vi "Needle Valve labVIEW Code.vi"() -> ()   [LabVIEW 2025]
uses:
  PIDController/PIDController.lvclass
  spikeController/spikeController.lvclass
  ControllerModeEnum.ctl
  modesEnum.ctl
  PIDController/PIDController.lvclass/PIDController.ctl
  0285ecf2-4d18-4427-ace1-61b1951a0741.vi
  d3b0afdc-d7ac-4f1a-8ecc-0aeb21fe1e80.vi
  c8945bc9-af31-4a2e-9b52-27840c61c0f1.vi
  e7797c04-791b-4eea-89a1-5a3bec2431d3.vi
  bf5fd3a0-ddf8-478e-bb95-a39885d33854.vi
  0890acf7-df83-934e-a7ac-ae51bc85d557.vi
  d872897a-af24-4a4d-87bc-a1bb59a840a8.vi
  <vilib>/Instr/_visa.llb/VISA Configure Serial Port (Instr).vi
  PIDController/updateLastValues.vi
  <vilib>/Utility/file.llb/Write Delimited Spreadsheet (string).vi
  <vilib>/Utility/file.llb/Read Delimited Spreadsheet (DBL).vi
  <vilib>/gmath/NI_Gmath.lvlib
  <vilib>/ptbypt/NI_PtbyPt.lvlib
panel:
  out "Motor Response":string
  in  "Disconnect":bool
  in  "Connect":bool
  in  "Use Dummy Data":bool
  in  "Reset":bool
  out "Reading Pressure Sensor 2":dbl(graph)
  out "PID Output 2":dbl(graph)
  out "the setted point":dbl
  out "the set position":dbl
  out "auto k_d":dbl
  out "auto k_i":dbl
  out "auto k_p":dbl
  out "spike str":string
  out "Array-to-save Pressure":string[][](array[string])
  out "Array-to-save PID":string[][](array[string])
  out "Array-to-save Spike":string[][](array[string])
  out "Array-to-save":string[][](array[string])
  out "to save":path
  out "Time Elapsed":dbl
  out "cycles_run":i32
  out "Autotune":bool
  in  "dt":dbl
  in  "tuning_rule":i32
  in  "min_cycles":i32
  in  "hysteresis":dbl
  in  "relay_amplitude":dbl
  in  "Exit Autotune":bool
  in  "AutoTune PID Params":bool
  out "last error":dbl
  in  "Use D1":bool
  in  "Use D2":bool
  in  "Use Avg":bool
  in  "Save Graphs":bool
  in  "Set setPoint":dbl format="%.3f"
  in  "Set Spike Position":dbl format="%.3f"
  in  "setPoint":dbl(knob) scale=0.0..1000.0
  in  "A_max":dbl=6.5
  in  "A_min":dbl
  in  "k_i":dbl
  in  "k_d":dbl
  in  "k_p":dbl
  out "SafetyClose":bool
  out "PID":bool
  out "Manual":bool
  out "Idle":bool
  out "Ducer1":bool
  out "Ducer2":bool
  out "Avg Ducers":bool
  out "Read Pressure Ducer":dbl
  out "Raw Pressure Ducer 2":dbl
  in  "spikeController.lvclass":refnum<class "spikeController.lvclass">
  out "underAmin":bool
  out "overAmax":bool
  out "PID Output":dbl[](graph)
  out "PID Translated Output":dbl
  out "PID Raw Output":dbl
  in  "loop stop 2":bool
  in  "loop stop 1":bool
  in  "PIDController.lvclass":refnum<class "PIDController.lvclass">
  out "VISA resource name out":refnum<visa-resource-name>
  in  "?":u32(colorbox)=16777225
  out "Reading Pressure Sensor":dbl[](graph)
  in  "?":dbl
  out "Motor Signal":string
  in  "stop program":bool
  in  "return spike":bool
  out "Spike Position \n(via Potentiometer)":dbl[](graph)
  out "Arduino Error":errorcluster
  in  "VISA resource Port":refnum<visa-resource-name>
  out "distance to go":dbl caption="Distance to Go (in)\n(For Reference Only)" format="%.3f"
  out "spike position":dbl format="%.3f"
  in  "Set Spike Position (in)":dbl(slide) scale=0.1..6.6
  out "?":dbl(slide) scale=0.0..1000.0
  out "Stagnation Flow Temp (K)\n(For Refrence only)":dbl
  out "Raw Pressure Ducer":dbl
  in  "Sensor Offsets":dbl[](array[numeric])=[10.0, 10.0, 0.0, 22.0]
  in  "Sensor K-values":dbl[](array[numeric])=[10.0, 10.0, 0.0, 22.0]
  in  "Exit PID Mode":bool
  in  "manual exit button":bool
  in  "Motor Control Loop Rate (ms)":dbl
  out "Set Motor RPM":dbl(knob) scale=0.0..200.0
  in  "PID Mode":bool
  in  "Manual Positioning Mode":bool
  in  "Stop Sensors":bool
  in  "Sensor Loop Rate (ms)":dbl
  out "Time Since Start (s)\n(For Reference Only)":dbl format="%.2f"
  in  "Start Sensors":bool
  in  "Load Inputs":bool
  in  "Save Inputs":bool
  out "Potentiometer distance":dbl
  out "Port":i32
  out "ConnectionType":i32
  out "DeviceType":i32
  out "Labjack error":errorcluster
  # "34HS59-6004S Motor Torque Curve (For Reference)"
  # "Labjack/Arduino Resources"
  # "Inputs and LabJack Sensor Monitors"
  # "PID Inputs"
  # "Motor RPM >200 RPM"
  # "Potentiometer"
  # "Inefficent Torque for High Mass Flow/Thrust Tests"
  # "Ducer"
  # "Thermocouple"
  # "<-- Uses same setpoint"
  # "Motor RPM < 200 RPM"
  # "(Labjack Auto-Populates)"
  # "(dial indicator for range reference)"
  # "COM Port for Arduino"
  # "Stop sensors automatically saves sensor data"
  # "Needliest"
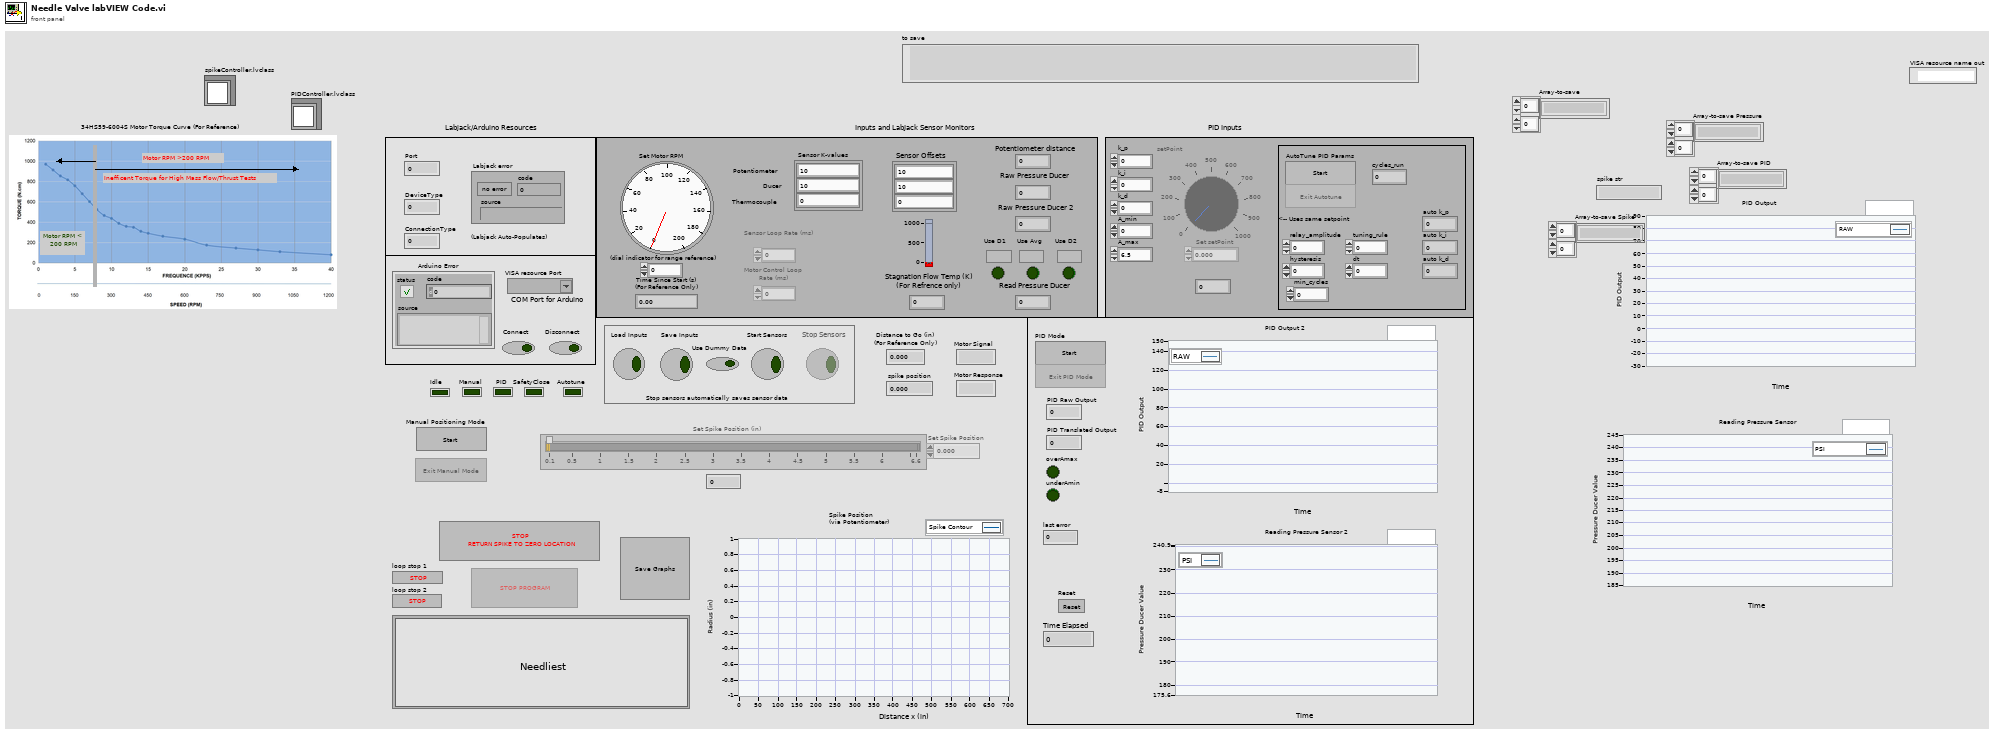
[diagram p1: front panel]
types:
  T1 = typedef "ControllerModeEnum.ctl" = enum16{"", "startControllers", "IdleControllers"}
  T2 = typedef "modesEnum.ctl" = enum16{"relay_autotune", "SafetyOpen", "SafetyClose", "SaveFile", "PIDControl", "ManualControl", "Idle"}
  T3 = enum8{"Enabled", "Disabled", "Disabled and Grayed Out"}
  T4 = enum16{"Potentiometer", "Ducer", "Thermocouple", "Ducer2"}
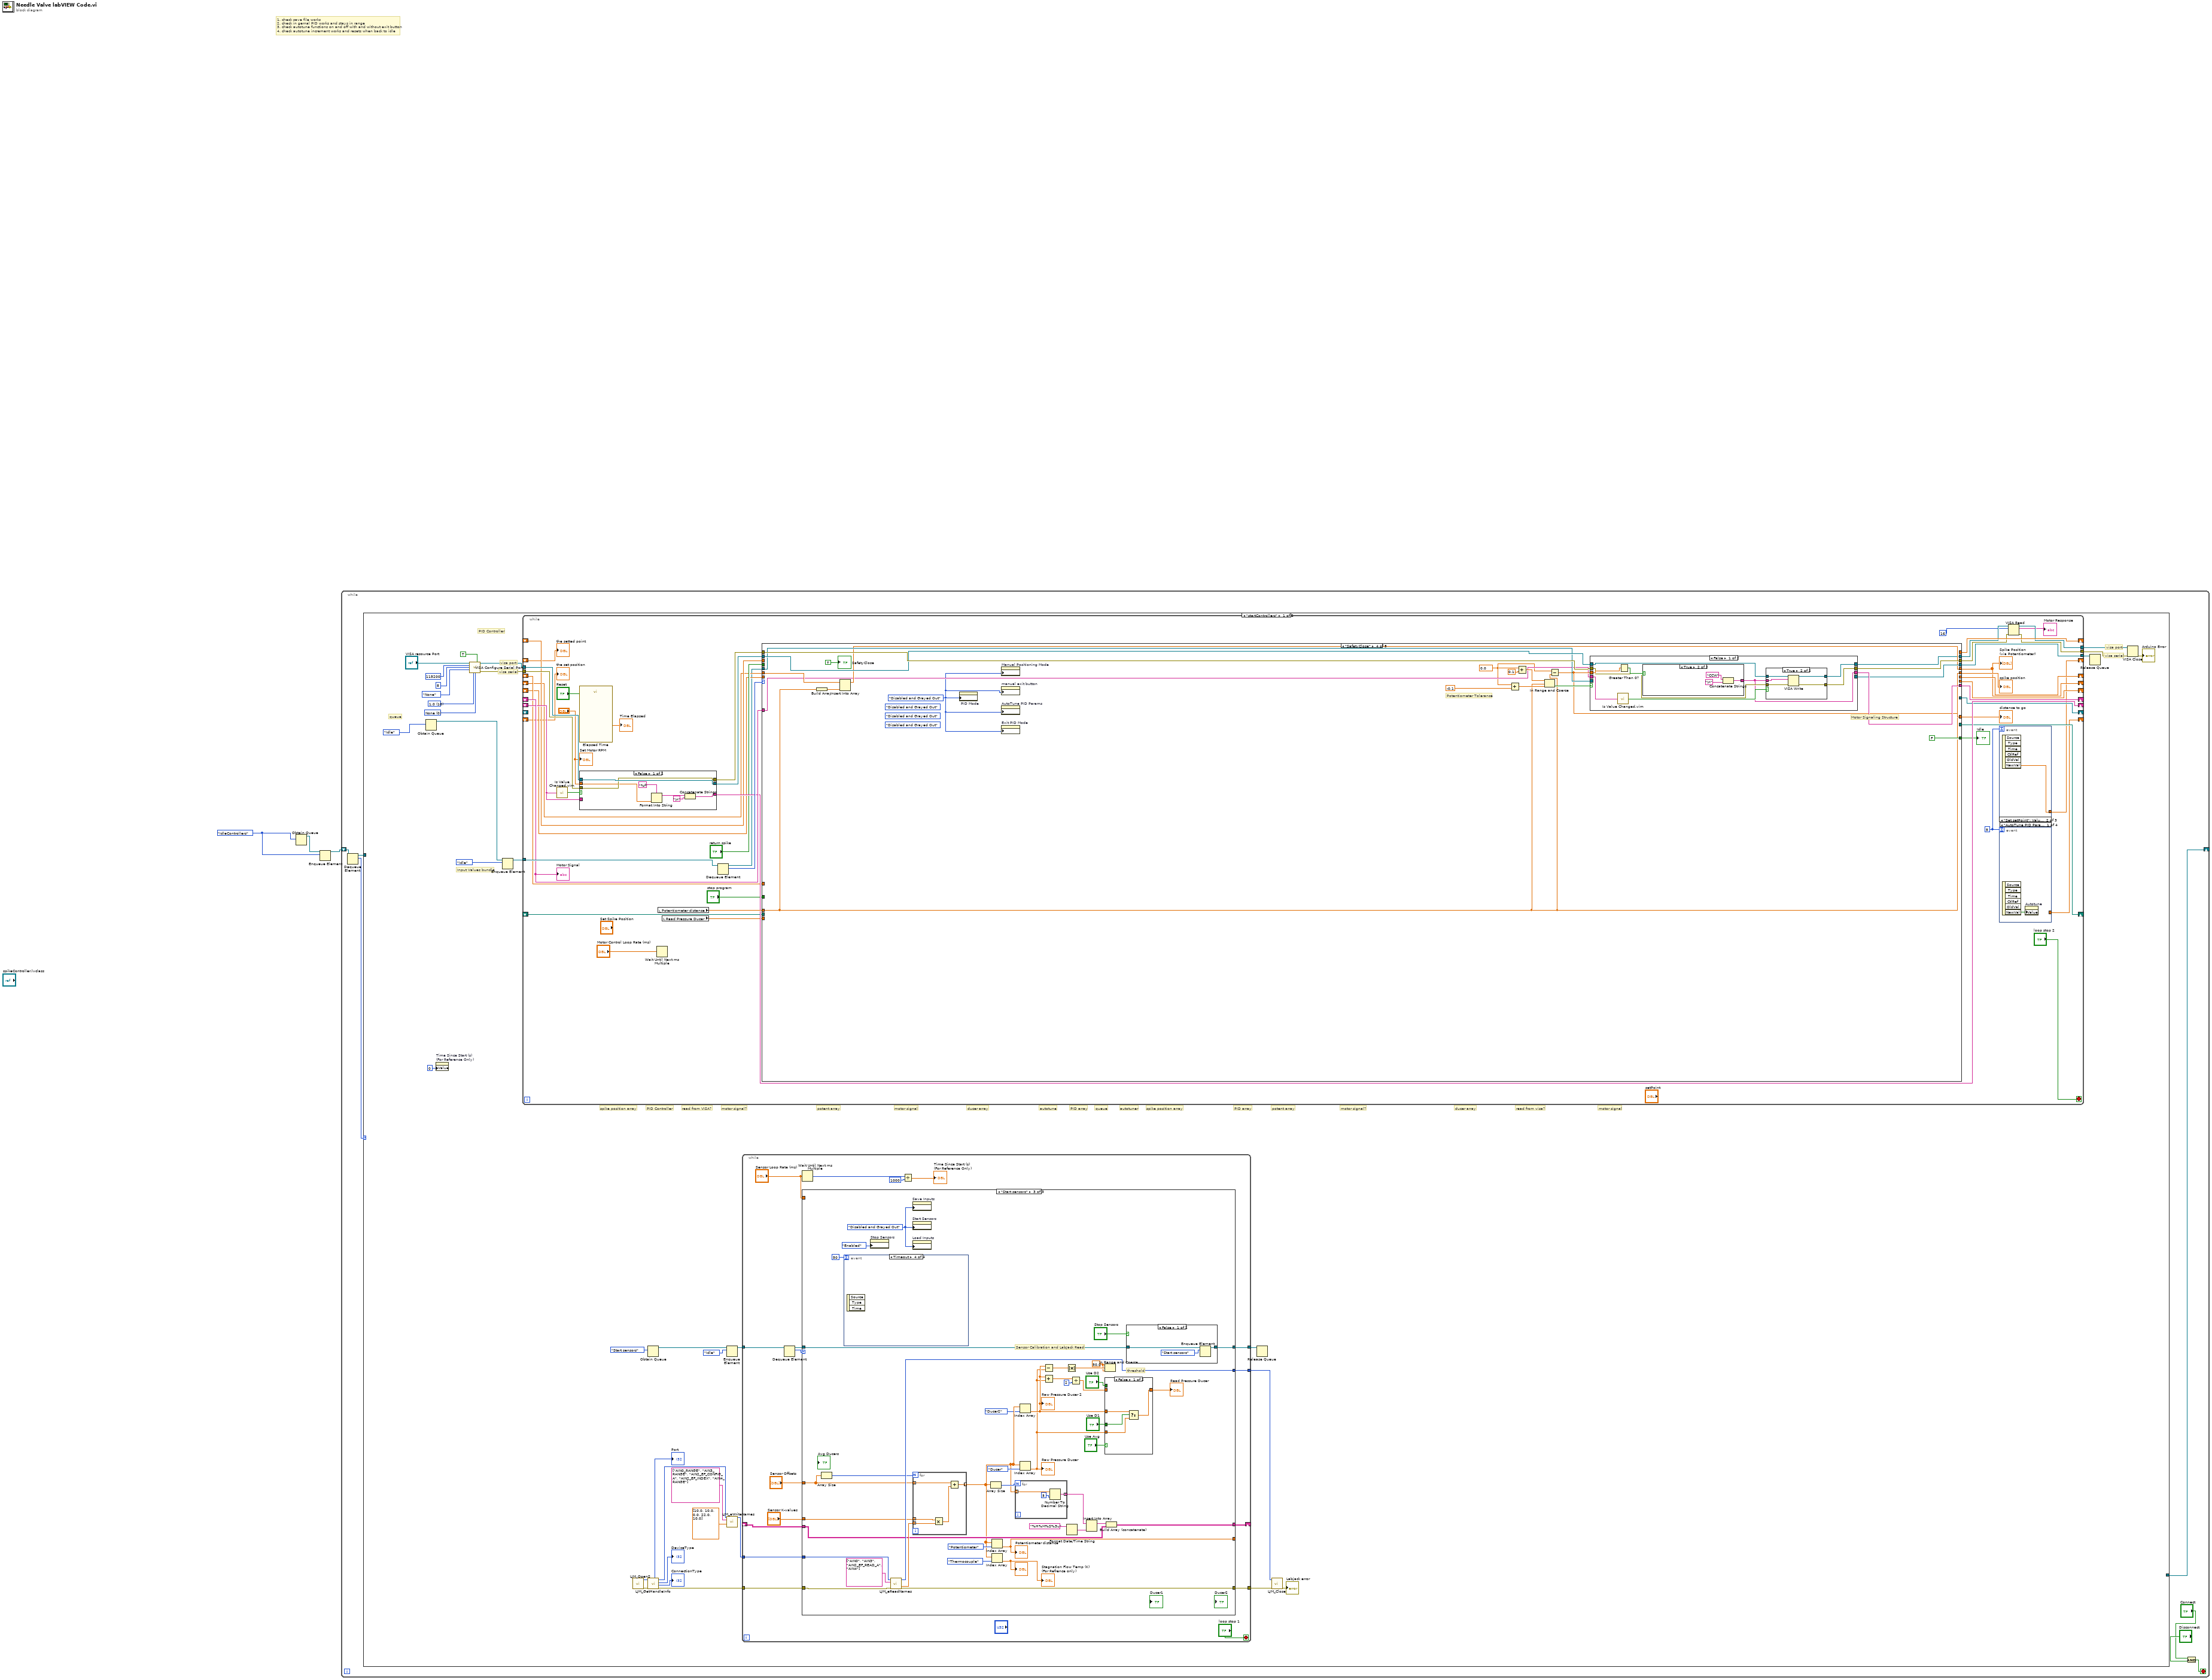
[diagram p0: block diagram]
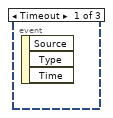
[diagram p2: hidden frame]
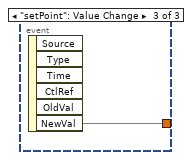
[diagram p3: hidden frame]
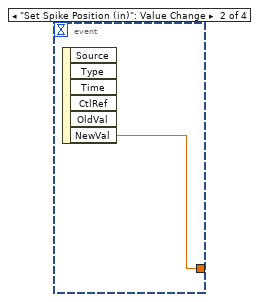
[diagram p4: hidden frame]
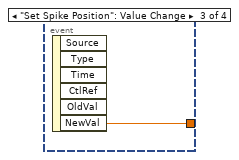
[diagram p5: hidden frame]
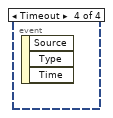
[diagram p6: hidden frame]
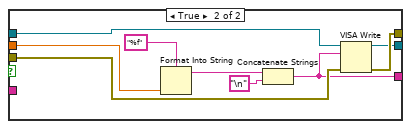
[diagram p7: hidden frame]
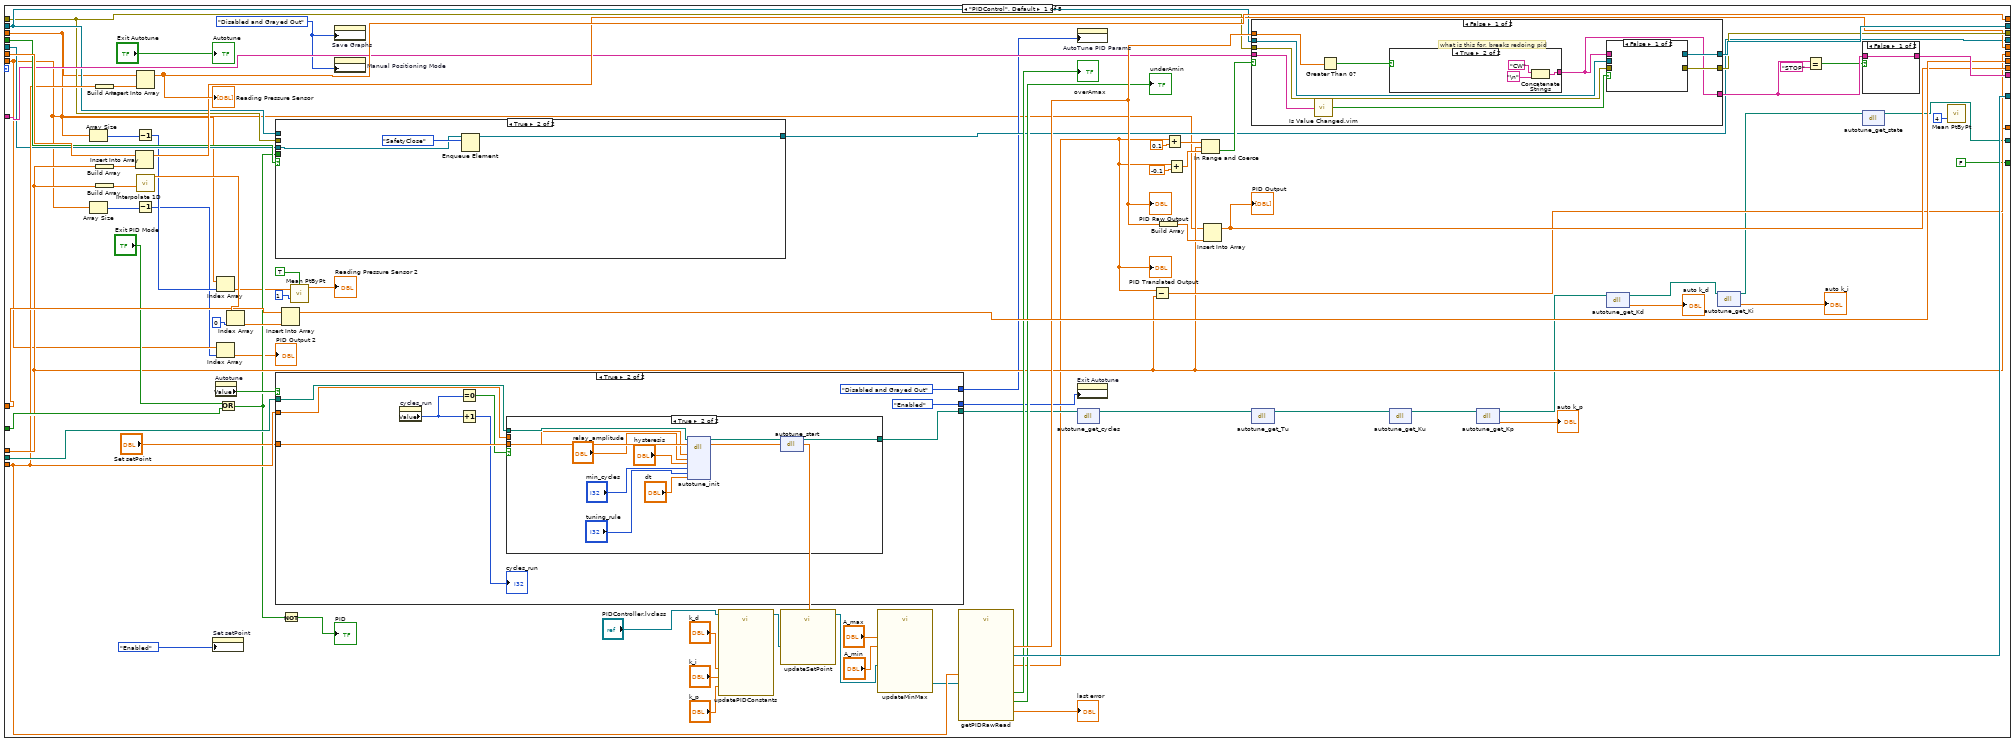
[diagram p8: hidden frame]
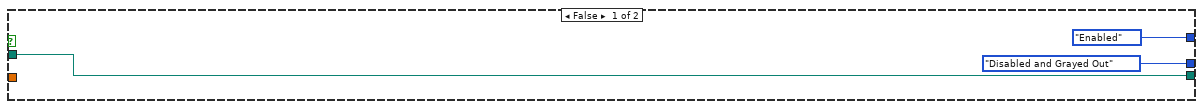
[diagram p9: hidden frame]
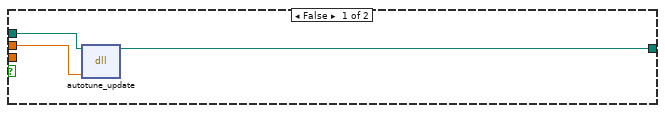
[diagram p10: hidden frame]
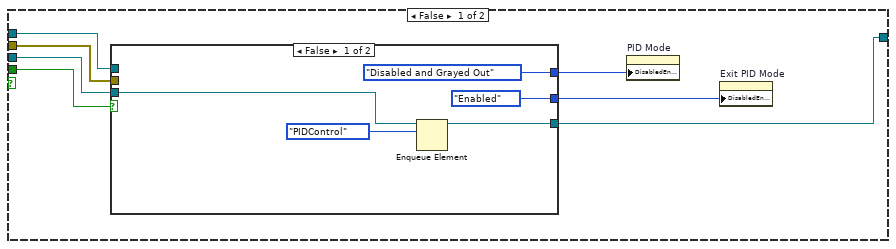
[diagram p11: hidden frame]
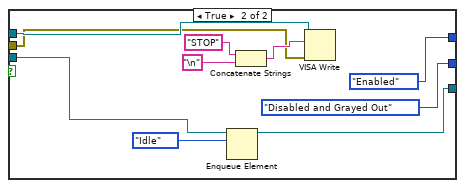
[diagram p12: hidden frame]
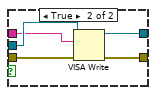
[diagram p14: hidden frame]
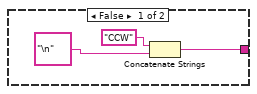
[diagram p15: hidden frame]
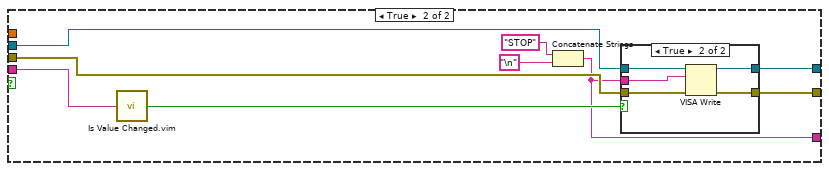
[diagram p16: hidden frame]
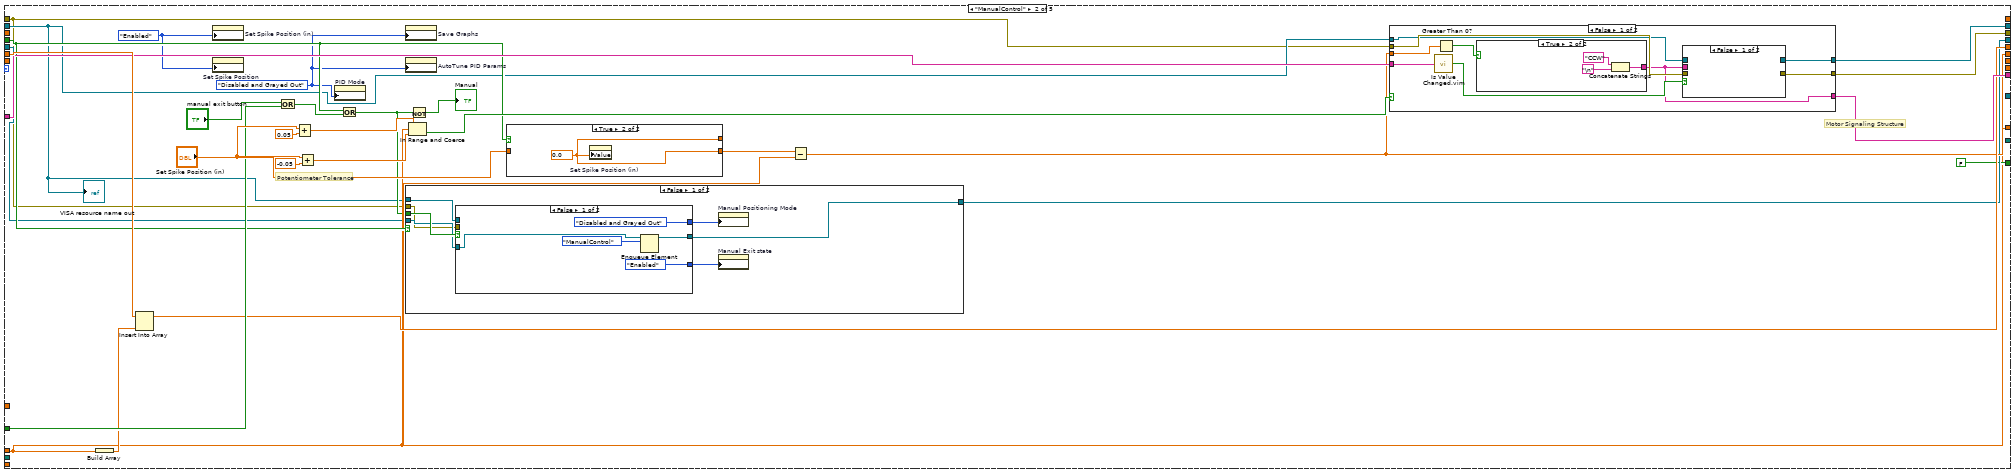
[diagram p18: hidden frame]
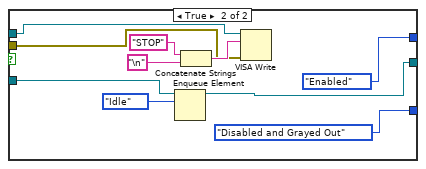
[diagram p19: hidden frame]
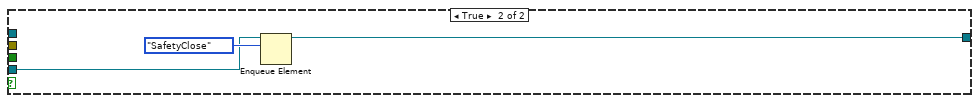
[diagram p20: hidden frame]
diagram:
  w2 = ControllerModeEnum."IdleControllers" ("ControllerModeEnum")
  # "1. check save file works\n2. check in gernal PID works and stays in range\n3. check autotune functions on and off with and without exit button\n4. check autotune increment works and resets when back to idle"
  n1 = Obtain Queue(element data type=w2) -> (queue out=w3:refnum<queue>)  [unwired: 4 in, 2 out]
  n2 = Enqueue Element(queue=w3, element=w2) -> (queue out=w1:refnum<queue>)  [unwired: 2 in, 2 out]
  n3 = while {
    shift-right: [w6] -> _
    shift-left: w1 -> [w4]
    stop <- w8 stop-if-true
    n4 = Dequeue Element(queue=w4) -> (queue out=w5:refnum<queue>, element=w7:T1)  [unwired: 2 in, 2 out]
    n5 = case shown="\"startControllers\"" w7 {
      tunnel: [_ w644] -> w6
      tunnel: w5 -> [_ w643]
      frame "startControllers" {
        w16 = u16 0 items=["None", "XON/XOFF", "RTS/CTS", "XON/XOFF & RTS/CTS", "DTR/DSR", "XON/XOFF & DTR/DSR"] ("flow control (0:none)")
        w17 = u16 10 items=["1.0"=10, "1.5"=15, "2.0"=20] ("stop bits (10: 1 bit)")
        # "PID Controller"
        # "PID Controller"
        # "spike position array"
        # "spike position array"
        # "motor signal"
        # "PID array"
        # "potent array"
        # "ducer array"
        # "motor signal?"
        # "read from visa?"
        # "visa serial"
        # "visa port"
        # "queue"
        # "queue"
        # "visa port"
        # "visa serial"
        # "autotuner"
        # "potent array"
        # "read from VISA?"
        # "ducer array"
        # "motor signal?"
        # "PID array"
        # "motor signal"
        # "autotune"
        # "Input Values bundle"
        n6 = Obtain Queue(element data type=modesEnum."Idle" ("modesEnum")) -> (queue out=w28:refnum<queue>)  [unwired: 4 in, 2 out]
        n7 = property on="Time Since Start (s)\n(For Reference Only)" class="DigNum (strict)"("Value"=u32 0 ("Time Since Start (s)\n(For Reference Only) 2")) -> ()  [unwired: 2 in, 2 out]
        n8 = call-poly "VISA Configure Serial Port"("VISA resource name"="VISA resource Port", "Enable Termination\nChar (T)"=TRUE ("Enable Termination\nChar (T)"), "baud rate (9600)"=u32 115200, "data bits (8)"=u16 8, "parity (0:none)"=enum16{"None", "Odd", "Even", "Mark", "Space"}."None", "stop bits (10: 1 bit)"=w17, "flow control (0:none)"=w16) -> ("VISA resource name out"=w14:refnum<visa-resource-name>, "error out"=w15:errorcluster)  [unwired: 7 in]
        n9 = Enqueue Element(queue=w28, element=modesEnum."Idle" ("modesEnum")) -> (queue out=w27:refnum<queue>)  [unwired: 2 in, 2 out]
        n10 = while {
          tunnel: w27 -> [w93]
          tunnel: [w91] -> w26
          tunnel: [w51] -> w22
          tunnel: [w48] -> w21
          shift-right: [w88] -> _
          shift-left: _ -> [w87]
          tunnel: w15 -> [w86]
          tunnel: w14 -> [w85]
          shift-right: [w81] -> _
          shift-left: _ -> [w80]
          shift-right: [w74] -> _
          shift-left: _ -> [_]
          shift-right: [w77] -> _
          shift-left: _ -> [w76]
          shift-right: [w75] -> _
          shift-left: _ -> [w72]
          shift-right: [w70] -> _
          shift-left: _ -> [w71]
          shift-right: [w56] -> _
          shift-left: _ -> [w68]
          shift-right: [w62] -> _
          shift-left: _ -> [w63]
          shift-right: [w58] -> _
          shift-left: _ -> [w59]
          shift-right: [w55] -> _
          shift-left: _ -> [w57]
          stop <- "loop stop 2" stop-if-true
          w54 = 5
          n11 = call "Is Value Changed.vim"("value"=w80) -> ("changed or first call?"=w82:bool)
          n12 = call "Elapsed Time"("Reset"="Reset") -> ("Elapsed Time (s)"=→"Time Elapsed":dbl)  [unwired: 11 in, 7 out]
          n13 = case shown="False" w82 {
            tunnel: w86 -> [w104 w114]
            tunnel: [w100 w106] -> w81
            tunnel: w85 -> [w105 w113]
            tunnel: [w104 w112] -> w84
            tunnel: [w105 w109] -> w83
            tunnel: "?" -> [w103 w111]
            tunnel: w80 -> [_ _]
            frame False {
              n14 = Format Into String(format string="%f", w103) -> (resulting string=w101:string)  [unwired: 2 in, 1 out]
              n15 = Concatenate Strings(w101, "\n" ("string")) -> (w100:string)
            }
            frame True {
              n16 = Format Into String(format string="%f", w111) -> (resulting string=w108:string)  [unwired: 2 in, 1 out]
              n17 = Concatenate Strings(w108, "\n" ("string")) -> (w106:string)
              n18 = VISA Write(VISA resource name=w113, write buffer=w106, error in (no error)=w114) -> (VISA resource name out=w109:refnum<visa-resource-name>, error out=w112:errorcluster)  [unwired: 1 out]
            }
          }
          n19 = Wait Until Next ms Multiple(millisecond multiple="Motor Control Loop Rate (ms)") -> ()  [unwired: 1 out]
          n20 = local read "Potentiometer distance"() -> (w89:dbl)
          n21 = local read "Read Pressure Ducer"() -> (w64:dbl)
          n22 = Dequeue Element(queue=w93) -> (queue out=w66:refnum<queue>, element=w92:T2)  [unwired: 2 in, 2 out]
          n23 = case shown="\"SafetyClose\"" w92 {
            tunnel: [w167 w294 w375 w417 _] -> w91
            tunnel: w66 -> [w133 w287 w376 w416 _]
            tunnel: w89 -> [w165 w289 _ w407 _]
            tunnel: w83 -> [w132 w286 w384 w420 _]
            tunnel: [w194 w307 w384 w406 _] -> w52
            tunnel: w84 -> [w131 w285 w383 w421 _]
            tunnel: [w193 w306 w383 w418 _] -> w49
            tunnel: [w189 w305 w382 w419 _] -> w88
            tunnel: w87 -> [w161 w297 w382 w412 _]
            tunnel: "return spike" -> [w166 w295 _ _ _]
            tunnel: [w183 _ _ _ _] -> w77
            tunnel: w76 -> [w184 _ _ _ _]
            tunnel: [w181 _ _ _ _] -> w75
            tunnel: w72 -> [w120 _ _ _ w481]
            tunnel: w64 -> [w159 _ _ _ _]
            tunnel: [w179 _ _ _ _] -> w74
            tunnel: w71 -> [w117 _ _ _ w480]
            tunnel: [w178 _ _ _ _] -> w70
            tunnel: "stop program" -> [w172 w302 _ _ _]
            tunnel: w68 -> [w170 w299 _ w415 w497]
            tunnel: [w169 w298 _ w414 _] -> w56
            tunnel: [w168 w296 _ w413 _] -> w67
            tunnel: [w165 w289 _ w407 _] -> w60
            tunnel: [FALSE FALSE TRUE FALSE FALSE] -> w65
            tunnel: w63 -> [w160 _ _ _ _]
            tunnel: [w148 _ _ _ _] -> w62
            frame "PIDControl", Default {
              w137 = T3."Disabled and Grayed Out" ("Disabled")
              n24 = Array Size(array=w120) -> (size(s)=w119:i32)
              n25 = Array Size(array=w117) -> (size(s)=w116:i32)
              n26 = Build Array(w159) -> (w182:dbl[])
              n27 = Build Array(w165) -> (w171:dbl[])
              n28 = Build Array(w165) -> (w187:dbl[])
              n29 = Insert Into Array(array=w170, new element=w171) -> (w169:dbl[])  [unwired: 1 in]
              n30 = Insert Into Array(array=w120, new element=w182) -> (w181:dbl[])  [unwired: 1 in]
              "Reading Pressure Sensor" <- w181
              n31 = Decrement(x=w119) -> (x-1=w118:i32)
              n32 = call <vilib>:"Interpolate 1D.vi"("xi"=w187) -> ("yi"=w186:dbl[])  [unwired: 8 in, 2 out]
              n33 = Decrement(x=w116) -> (x-1=w115:i32)
              n34 = property on="Set setPoint" class="DigNum (strict)"("DisabledEnum"=T3."Enabled" ("Disabled")) -> ()  [unwired: 2 in, 2 out]
              n35 = property on="Autotune" class="Bool (strict)"() -> ("Value"=w158:bool)  [unwired: 2 in, 2 out]
              n36 = Index Array(array=w120, index=w118) -> (element=w124:dbl)
              n37 = Index Array(array=w117, index=w115) -> (element=→"PID Output 2":dbl)
              n38 = Or(x="Exit PID Mode", y=w172) -> (x .or. y?=w134:bool)
              n39 = Index Array(array=w186, index=0) -> (element=w180:dbl)
              n40 = case shown="True" w166 {
                tunnel: [w225 w247] -> w167
                tunnel: w134 -> [w229 _]
                tunnel: w133 -> [w228 w245]
                tunnel: w132 -> [w227 _]
                tunnel: w131 -> [w226 _]
                frame False {
                  n41 = case shown="False" w229 {
                    tunnel: w228 -> [w234 w244]
                    tunnel: [w233 w243] -> w225
                    tunnel: w227 -> [_ w239]
                    tunnel: w226 -> [_ w238]
                    tunnel: [T3."Disabled and Grayed Out" ("Disabled") T3."Enabled" ("Disabled")] -> w224
                    tunnel: [T3."Enabled" ("Disabled") T3."Disabled and Grayed Out" ("Disabled")] -> w223
                    frame False {
                      n42 = Enqueue Element(queue=w234, element=modesEnum."PIDControl" ("modesEnum")) -> (queue out=w233:refnum<queue>)  [unwired: 2 in, 2 out]
                    }
                    frame True {
                      n43 = Enqueue Element(queue=w244, element=modesEnum."Idle" ("modesEnum")) -> (queue out=w243:refnum<queue>)  [unwired: 2 in, 2 out]
                      n44 = Concatenate Strings("STOP" ("write buffer"), "\n" ("write buffer")) -> (w242:string)
                      n45 = VISA Write(VISA resource name=w239, write buffer=w242, error in (no error)=w238) -> ()  [unwired: 3 out]
                    }
                  }
                  n46 = property on="PID Mode" class="Bool"("DisabledEnum"=w224) -> ()  [unwired: 2 in, 2 out]
                  n47 = property on="Exit PID Mode" class="Bool"("DisabledEnum"=w223) -> ()  [unwired: 2 in, 2 out]
                }
                frame True {
                  n48 = Enqueue Element(queue=w245, element=modesEnum."SafetyClose" ("modesEnum")) -> (queue out=w247:refnum<queue>)  [unwired: 2 in, 2 out]
                }
              }
              n49 = case shown="True" w158 {
                tunnel: w160 -> [w201 w208]
                tunnel: [w201 w207] -> w149
                tunnel: w159 -> [_ w206]
                tunnel: [T3."Disabled and Grayed Out" ("Disabled") T3."Enabled" ("Disabled")] -> w157
                tunnel: [T3."Enabled" ("Disabled") T3."Disabled and Grayed Out" ("Disabled")] -> w156
                tunnel: "Set setPoint" -> [_ w202]
                frame False {
                }
                frame True {
                  n50 = property on="cycles_run" class="DigNum (strict)"() -> ("Value"=w210:i32)  [unwired: 2 in, 2 out]
                  n51 = Equal To 0?(x=w210) -> (x = 0?=w205:bool)
                  n52 = Increment(x=w210) -> (x+1=→"cycles_run":i32)
                  n53 = case shown="True" w205 {
                    tunnel: w208 -> [w213 w222]
                    tunnel: [w212 w220] -> w207
                    tunnel: w206 -> [w211 _]
                    tunnel: w202 -> [_ w214]
                    frame False {
                      n54 = dll-call lib="Users/alexpoulin/Downloads/git/needliest/labview/relay_autotune_library/relay_autotune.dylib" fn="autotune_update"(path in=w213, "pv"=w211) -> (path out=w212:path)  [unwired: 4 in, 1 out]
                    }
                    frame True {
                      n55 = dll-call lib="Users/alexpoulin/Downloads/git/needliest/labview/relay_autotune_library/relay_autotune.dylib" fn="autotune_init"(path in=w222, "setpoint"=w214, "relay_amplitude"="relay_amplitude", "hysteresis"="hysteresis", "min_cycles"="min_cycles", "tuning_rule"="tuning_rule", "dt"="dt") -> (path out=w221:path)  [unwired: 9 in, 1 out]
                      n56 = dll-call lib="Users/alexpoulin/Downloads/git/needliest/labview/relay_autotune_library/relay_autotune.dylib" fn="autotune_start"(path in=w221) -> (path out=w220:path)  [unwired: 3 in, 1 out]
                    }
                  }
                }
              }
              n57 = Insert Into Array(array=w184, new element=w180) -> (w183:dbl[])  [unwired: 1 in]
              n58 = Not(x=w134) -> (.not. x?=→"PID":bool)
              n59 = call <vilib>:"Mean PtByPt.vi"("x"=w124, "sample length"=1, "initialize"=TRUE) -> ("mean"=→"Reading Pressure Sensor 2":dbl)  [unwired: 1 in, 1 out]
              n60 = property on="Save Graphs" class="Bool"("DisabledEnum"=w137) -> ()  [unwired: 2 in, 2 out]
              n61 = property on="Manual Positioning Mode" class="Bool"("DisabledEnum"=w137) -> ()  [unwired: 2 in, 2 out]
              n62 = call "updatePIDConstants.vi"("new k_d"="k_d", "new k_p"="k_p", "new k_i"="k_i", "PIDController in"="PIDController.lvclass") -> ("PIDController out"=w141:refnum<class "PIDController.lvclass">)  [unwired: 6 in, 1 out]
              n63 = call "updateSetPoint.vi"("new setpoint"="Set setPoint", "PIDController in"=w141) -> ("PIDController out"=w140:refnum<class "PIDController.lvclass">)  [unwired: 8 in, 1 out]
              n64 = call "updateMinMax.vi"("a_max"="A_max", "a_min"="A_min", "PIDController in"=w140) -> ("PIDController out"=w139:refnum<class "PIDController.lvclass">)  [unwired: 7 in, 1 out]
              n65 = call "getPIDRawRead.vi"("sensorValue"=w159, "PIDController in"=w139) -> ("overAmin"=→"underAmin":bool, "translatedPIDOutput"=w135:dbl, "PIDRawRead"=w177:dbl, "PIDController out"=w179:refnum<class "PIDController.lvclass">, "underAmax"=→"overAmax":bool, "lastErrorRead"=→"last error":dbl)  [unwired: 4 in]
              "PID Raw Output" <- w177
              "PID Translated Output" <- w135
              n66 = property on="AutoTune PID Params" class="Bool"("DisabledEnum"=w156) -> ()  [unwired: 2 in, 2 out]
              n67 = property on="Exit Autotune" class="Bool"("DisabledEnum"=w157) -> ()  [unwired: 2 in, 2 out]
              n68 = dll-call lib="Users/alexpoulin/Downloads/git/needliest/labview/relay_autotune_library/relay_autotune.dylib" fn="autotune_get_cycles"(path in=w149) -> (path out=w155:path)  [unwired: 3 in, 1 out]
              n69 = Subtract(x=w135, y=w165) -> (x-y=w168:dbl)
              n70 = Build Array(w177) -> (w176:dbl[])
              n71 = Add(x=w135, y=0.1) -> (x+y=w198:dbl)
              n72 = Add(x=w135, y=-0.1) -> (x+y=w196:dbl)
              n73 = In Range and Coerce(upper limit=w198, x=w165, lower limit=w196) -> (In Range?=w192:bool)  [unwired: 1 out]
              n74 = Insert Into Array(array=w117, new element=w176) -> (w178:dbl[])  [unwired: 1 in]
              "PID Output" <- w178
              n75 = case shown="False" w192 {
                tunnel: w177 -> [w257 _]
                tunnel: w132 -> [w255 w278]
                tunnel: [w253 w275] -> w194
                tunnel: w131 -> [w256 w274]
                tunnel: [w254 w273] -> w193
                tunnel: [w250 w270] -> w190
                tunnel: w161 -> [w252 w277]
                frame False {
                  # "what is this for, breaks redoing pid"
                  n76 = call "Is Value Changed.vim"("value"=w252) -> ("changed or first call?"=w251:bool)
                  n77 = Greater Than 0?(x=w257) -> (x > 0?=w258:bool)
                  n78 = case shown="True" w258 {
                    tunnel: [w264 w267] -> w250
                    frame False {
                      n79 = Concatenate Strings("CCW" ("write buffer"), "\n" ("write buffer")) -> (w264:string)
                    }
                    frame True {
                      n80 = Concatenate Strings("CW" ("write buffer"), "\n" ("write buffer")) -> (w267:string)
                    }
                  }
                  n81 = case shown="False" w251 {
                    tunnel: w256 -> [_ w263]
                    tunnel: w255 -> [_ w262]
                    tunnel: [_ w261] -> w254
                    tunnel: [_ w260] -> w253
                    tunnel: w250 -> [_ w259]
                    frame False {
                    }
                    frame True {
                      n82 = VISA Write(VISA resource name=w262, write buffer=w259, error in (no error)=w263) -> (VISA resource name out=w260:refnum<visa-resource-name>, error out=w261:errorcluster)  [unwired: 1 out]
                    }
                  }
                }
                frame True {
                  n83 = call "Is Value Changed.vim"("value"=w277) -> ("changed or first call?"=w276:bool)
                  n84 = Concatenate Strings("STOP" ("write buffer"), "\n" ("write buffer")) -> (w270:string)
                  n85 = case shown="True" w276 {
                    tunnel: w270 -> [_ w283]
                    tunnel: w278 -> [_ w282]
                    tunnel: [_ w281] -> w275
                    tunnel: w274 -> [_ w280]
                    tunnel: [_ w279] -> w273
                    frame False {
                    }
                    frame True {
                      n86 = VISA Write(VISA resource name=w282, write buffer=w283, error in (no error)=w280) -> (VISA resource name out=w281:refnum<visa-resource-name>, error out=w279:errorcluster)  [unwired: 1 out]
                    }
                  }
                }
              }
              n87 = dll-call lib="Users/alexpoulin/Downloads/git/needliest/labview/relay_autotune_library/relay_autotune.dylib" fn="autotune_get_Tu"(path in=w155) -> (path out=w154:path)  [unwired: 3 in, 1 out]
              n88 = dll-call lib="Users/alexpoulin/Downloads/git/needliest/labview/relay_autotune_library/relay_autotune.dylib" fn="autotune_get_Ku"(path in=w154) -> (path out=w153:path)  [unwired: 3 in, 1 out]
              n89 = dll-call lib="Users/alexpoulin/Downloads/git/needliest/labview/relay_autotune_library/relay_autotune.dylib" fn="autotune_get_Kp"(path in=w153) -> (path out=w152:path, "g_ctx.Kp"=→"auto k_p":dbl)  [unwired: 2 in, 1 out]
              n90 = dll-call lib="Users/alexpoulin/Downloads/git/needliest/labview/relay_autotune_library/relay_autotune.dylib" fn="autotune_get_Kd"(path in=w152) -> (path out=w151:path, "g_ctx.Kd"=→"auto k_d":dbl)  [unwired: 2 in, 1 out]
              n91 = dll-call lib="Users/alexpoulin/Downloads/git/needliest/labview/relay_autotune_library/relay_autotune.dylib" fn="autotune_get_Ki"(path in=w151) -> (path out=w150:path, "g_ctx.Ki"=→"auto k_i":dbl)  [unwired: 2 in, 1 out]
              n92 = Equal?(x=w190, y="STOP" ("write buffer")) -> (x = y?=w188:bool)
              n93 = case shown="False" w188 {
                tunnel: [w248 w249] -> w189
                tunnel: w190 -> [w248 w249]
                frame False {
                }
                frame True {
                }
              }
              n94 = dll-call lib="Users/alexpoulin/Downloads/git/needliest/labview/relay_autotune_library/relay_autotune.dylib" fn="autotune_get_state"(path in=w150) -> (path out=w148:path)  [unwired: 3 in, 1 out]
              n95 = call <vilib>:"Mean PtByPt.vi"("sample length"=4) -> ()  [unwired: 3 in, 2 out]
              "Autotune" <- "Exit Autotune"
            }
            frame "ManualControl" {
              w284 = T3."Enabled" ("Disabled")
              w290 = T3."Disabled and Grayed Out" ("Disabled")
              # "Motor Signaling Structure"
              # "Potentiometer Tolerance"
              n96 = Build Array(w289) -> (w300:dbl[])
              n97 = Insert Into Array(array=w299, new element=w300) -> (w298:dbl[])  [unwired: 1 in]
              n98 = property on="Set Spike Position (in)" class="Slide (strict)"("DisabledEnum"=w284) -> ()  [unwired: 2 in, 2 out]
              n99 = property on="Set Spike Position" class="DigNum (strict)"("DisabledEnum"=w284) -> ()  [unwired: 2 in, 2 out]
              n100 = Or(x="manual exit button", y=w302) -> (x .or. y?=w301:bool)
              n101 = Add(x="Set Spike Position (in)", y=0.05) -> (x+y=w311:dbl)
              n102 = Add(x="Set Spike Position (in)", y=-0.05) -> (x+y=w309:dbl)
              n103 = property on="PID Mode" class="Bool"("DisabledEnum"=w290) -> ()  [unwired: 2 in, 2 out]
              n104 = Or(x=w295, y=w301) -> (x .or. y?=w288:bool)
              n105 = property on="Save Graphs" class="Bool"("DisabledEnum"=w290) -> ()  [unwired: 2 in, 2 out]
              n106 = property on="AutoTune PID Params" class="Bool"("DisabledEnum"=w290) -> ()  [unwired: 2 in, 2 out]
              n107 = case shown="False" w295 {
                tunnel: [w315 w337] -> w294
                tunnel: w288 -> [w319 _]
                tunnel: w287 -> [w318 w335]
                tunnel: w286 -> [w317 _]
                tunnel: w285 -> [w316 _]
                frame False {
                  n108 = case shown="False" w319 {
                    tunnel: w318 -> [w324 w334]
                    tunnel: [w323 w333] -> w315
                    tunnel: w317 -> [_ w329]
                    tunnel: w316 -> [_ w328]
                    tunnel: [T3."Enabled" ("Disabled") T3."Disabled and Grayed Out" ("Disabled")] -> w314
                    tunnel: [T3."Disabled and Grayed Out" ("Disabled") T3."Enabled" ("Disabled")] -> w313
                    frame False {
                      n109 = Enqueue Element(queue=w324, element=modesEnum."ManualControl" ("modesEnum")) -> (queue out=w323:refnum<queue>)  [unwired: 2 in, 2 out]
                    }
                    frame True {
                      n110 = Enqueue Element(queue=w334, element=modesEnum."Idle" ("modesEnum")) -> (queue out=w333:refnum<queue>)  [unwired: 2 in, 2 out]
                      n111 = Concatenate Strings("STOP" ("write buffer"), "\n" ("write buffer")) -> (w332:string)
                      n112 = VISA Write(VISA resource name=w329, write buffer=w332, error in (no error)=w328) -> ()  [unwired: 3 out]
                    }
                  }
                  n113 = property on="Manual Positioning Mode" class="Bool"("DisabledEnum"=w313) -> ()  [unwired: 2 in, 2 out]
                  n114 = property on="Manual Exit state" class="Bool"("DisabledEnum"=w314) -> ()  [unwired: 2 in, 2 out]
                }
                frame True {
                  n115 = Enqueue Element(queue=w335, element=modesEnum."SafetyClose" ("modesEnum")) -> (queue out=w337:refnum<queue>)  [unwired: 2 in, 2 out]
                }
              }
              n116 = In Range and Coerce(upper limit=w311, x=w289, lower limit=w309) -> (In Range?=w312:bool)  [unwired: 1 out]
              n117 = Not(x=w288) -> (.not. x?=→"Manual":bool)
              n118 = case shown="True" w295 {
                tunnel: [w338 w339] -> w293
                tunnel: "Set Spike Position (in)" -> [w338 _]
                tunnel: [w338 w339] -> _
                frame False {
                }
                frame True {
                  w339 = 0.0
                  n119 = property on="Set Spike Position (in)" class="Slide (strict)"("Value"=w339) -> ()  [unwired: 2 in, 2 out]
                }
              }
              n120 = Subtract(x=w293, y=w289) -> (x-y=w296:dbl)
              n121 = case shown="False" w312 {
                tunnel: w296 -> [w347 _]
                tunnel: w286 -> [w345 w368]
                tunnel: [w343 w365] -> w307
                tunnel: w285 -> [w346 w364]
                tunnel: [w344 w363] -> w306
                tunnel: [w340 w360] -> w305
                tunnel: w297 -> [w342 w367]
                frame False {
                  n122 = call "Is Value Changed.vim"("value"=w342) -> ("changed or first call?"=w341:bool)
                  n123 = Greater Than 0?(x=w347) -> (x > 0?=w348:bool)
                  n124 = case shown="True" w348 {
                    tunnel: [w354 w357] -> w340
                    frame False {
                      n125 = Concatenate Strings("CW" ("write buffer"), "\n" ("write buffer")) -> (w354:string)
                    }
                    frame True {
                      n126 = Concatenate Strings("CCW" ("write buffer"), "\n" ("write buffer")) -> (w357:string)
                    }
                  }
                  n127 = case shown="False" w341 {
                    tunnel: w346 -> [_ w353]
                    tunnel: w345 -> [_ w352]
                    tunnel: [_ w351] -> w344
                    tunnel: [_ w350] -> w343
                    tunnel: w340 -> [_ w349]
                    frame False {
                    }
                    frame True {
                      n128 = VISA Write(VISA resource name=w352, write buffer=w349, error in (no error)=w353) -> (VISA resource name out=w350:refnum<visa-resource-name>, error out=w351:errorcluster)  [unwired: 1 out]
                    }
                  }
                }
                frame True {
                  n129 = call "Is Value Changed.vim"("value"=w367) -> ("changed or first call?"=w366:bool)
                  n130 = Concatenate Strings("STOP" ("write buffer"), "\n" ("write buffer")) -> (w360:string)
                  n131 = case shown="True" w366 {
                    tunnel: w360 -> [_ w373]
                    tunnel: w368 -> [_ w372]
                    tunnel: [_ w371] -> w365
                    tunnel: w364 -> [_ w370]
                    tunnel: [_ w369] -> w363
                    frame False {
                    }
                    frame True {
                      n132 = VISA Write(VISA resource name=w372, write buffer=w373, error in (no error)=w370) -> (VISA resource name out=w371:refnum<visa-resource-name>, error out=w369:errorcluster)  [unwired: 1 out]
                    }
                  }
                }
              }
              "VISA resource name out" <- w286
            }
            frame "Idle" {
              w374 = T3."Disabled and Grayed Out" ("Disabled")
              w380 = T3."Enabled" ("Disabled")
              n133 = event shown="[4] \"return spike\": Value Change" {
                selector: _ -> [_ _ _ _ _]
                dyn-events: _ -> [_ _ _ _ _]
                timeout: _ -> [_ _ _ _ _]
                tunnel: w376 -> [w392 w395 w398 w401 w403]
                tunnel: [w391 w394 w397 w400 w404] -> w375
                event "Manual Positioning Mode": Value Change {
                  n134 = event-data() -> ()  [unwired: 1 in, 6 out]
                  n135 = Enqueue Element(queue=w392, element=modesEnum."ManualControl" ("modesEnum")) -> (queue out=w391:refnum<queue>)  [unwired: 2 in, 2 out]
                }
                event "Save Graphs": Value Change {
                  n136 = event-data() -> ()  [unwired: 1 in, 6 out]
                  n137 = Enqueue Element(queue=w395, element=modesEnum."SaveFile" ("modesEnum")) -> (queue out=w394:refnum<queue>)  [unwired: 2 in, 2 out]
                }
                event "PID Mode": Value Change {
                  n138 = event-data() -> ()  [unwired: 1 in, 6 out]
                  n139 = Enqueue Element(queue=w398, element=modesEnum."PIDControl" ("modesEnum")) -> (queue out=w397:refnum<queue>)  [unwired: 2 in, 2 out]
                }
                event "AutoTune PID Params": Value Change {
                  n140 = event-data() -> ()  [unwired: 1 in, 6 out]
                  n141 = property on="cycles_run" class="DigNum (strict)"("Value"=0) -> ()  [unwired: 2 in, 2 out]
                  n142 = Enqueue Element(queue=w401, element=modesEnum."Idle" ("modesEnum")) -> (queue out=w400:refnum<queue>)  [unwired: 2 in, 2 out]
                }
                event "return spike": Value Change {
                  n143 = event-data() -> ()  [unwired: 1 in, 6 out]
                  n144 = Enqueue Element(queue=w403, element=modesEnum."SafetyClose" ("modesEnum")) -> (queue out=w404:refnum<queue>)  [unwired: 2 in, 2 out]
                }
              }
              n145 = property on="Idle" class="Bool (strict)"("Value"=TRUE) -> ()  [unwired: 2 in, 2 out]
              n146 = property on="SafetyClose" class="Bool (strict)"("Value"=FALSE) -> ()  [unwired: 2 in, 2 out]
              n147 = Concatenate Strings("STOP" ("write buffer"), "\n" ("write buffer")) -> (w387:string)
              n148 = VISA Write(VISA resource name=w384, write buffer=w387, error in (no error)=w383) -> ()  [unwired: 3 out]
              n149 = property on="AutoTune PID Params" class="Bool"("DisabledEnum"=T3."Enabled" ("Disabled")) -> ()  [unwired: 2 in, 2 out]
              n150 = property on="PID Mode" class="Bool"("DisabledEnum"=w380) -> ()  [unwired: 2 in, 2 out]
              n151 = property on="Manual Positioning Mode" class="Bool"("DisabledEnum"=w380) -> ()  [unwired: 2 in, 2 out]
              n152 = property on="Save Graphs" class="Bool"("DisabledEnum"=w380) -> ()  [unwired: 2 in, 2 out]
              n153 = property on="Set setPoint" class="DigNum (strict)"("DisabledEnum"=w374) -> ()  [unwired: 2 in, 2 out]
              n154 = property on="Set Spike Position" class="DigNum (strict)"("DisabledEnum"=w374) -> ()  [unwired: 2 in, 2 out]
              n155 = property on="Set Spike Position (in)" class="Slide (strict)"("DisabledEnum"=w374) -> ()  [unwired: 2 in, 2 out]
              n156 = property on="Exit Autotune" class="Bool"("DisabledEnum"=w374) -> ()  [unwired: 2 in, 2 out]
              n157 = property on="PID Exit" class="Bool"("DisabledEnum"=T3."Disabled and Grayed Out" ("Disabled")) -> ()  [unwired: 2 in, 2 out]
              n158 = property on="Manual Exit" class="Bool"("DisabledEnum"=T3."Disabled and Grayed Out" ("Disabled")) -> ()  [unwired: 2 in, 2 out]
            }
            frame "SafetyClose" {
              (unwired) T3."Disabled and Grayed Out" ("Disabled")
              (unwired) T3."Disabled and Grayed Out" ("Disabled")
              (unwired) T3."Disabled and Grayed Out" ("Disabled")
              w410 = T3."Disabled and Grayed Out" ("Disabled")
              w408 = 0.0
              # "Motor Signaling Structure"
              # "Potentiometer Tolerance"
              n159 = Build Array(w407) -> (w422:dbl[])
              n160 = Insert Into Array(array=w415, new element=w422) -> (w414:dbl[])  [unwired: 1 in]
              n161 = property on="PID Mode" class="Bool"("DisabledEnum"=w410) -> ()  [unwired: 2 in, 2 out]
              n162 = property on="Manual Positioning Mode" class="Bool"("DisabledEnum"=w410) -> ()  [unwired: 2 in, 2 out]
              n163 = property on="manual exit button" class="Bool"("DisabledEnum"=w410) -> ()  [unwired: 2 in, 2 out]
              n164 = property on="AutoTune PID Params" class="Bool"("DisabledEnum"=w410) -> ()  [unwired: 2 in, 2 out]
              n165 = property on="Exit PID Mode" class="Bool"("DisabledEnum"=w410) -> ()  [unwired: 2 in, 2 out]
              n166 = Add(x=w408, y=-0.1) -> (x+y=w424:dbl)
              n167 = Add(x=w408, y=0.1) -> (x+y=w426:dbl)
              n168 = In Range and Coerce(upper limit=w426, x=w407, lower limit=w424) -> (In Range?=w427:bool)  [unwired: 1 out]
              n169 = Subtract(x=w408, y=w407) -> (x-y=w413:dbl)
              n170 = case shown="False" w427 {
                tunnel: w413 -> [w435 _]
                tunnel: w420 -> [w433 w459]
                tunnel: [w431 w456] -> w406
                tunnel: w421 -> [w434 w455]
                tunnel: [w432 w454] -> w418
                tunnel: [w428 w451] -> w419
                tunnel: w412 -> [w430 w458]
                tunnel: w416 -> [_ w450]
                tunnel: [_ w449] -> w417
                frame False {
                  n171 = call "Is Value Changed.vim"("value"=w430) -> ("changed or first call?"=w429:bool)
                  n172 = Greater Than 0?(x=w435) -> (x > 0?=w436:bool)
                  n173 = case shown="True" w436 {
                    tunnel: [w442 w445] -> w428
                    frame False {
                      n174 = Concatenate Strings("CW" ("write buffer"), "\n" ("write buffer")) -> (w442:string)
                    }
                    frame True {
                      n175 = Concatenate Strings("CCW" ("write buffer"), "\n" ("write buffer")) -> (w445:string)
                    }
                  }
                  n176 = case shown="True" w429 {
                    tunnel: w434 -> [_ w441]
                    tunnel: w433 -> [_ w440]
                    tunnel: [_ w439] -> w432
                    tunnel: [_ w438] -> w431
                    tunnel: w428 -> [_ w437]
                    frame False {
                    }
                    frame True {
                      n177 = VISA Write(VISA resource name=w440, write buffer=w437, error in (no error)=w441) -> (VISA resource name out=w438:refnum<visa-resource-name>, error out=w439:errorcluster)  [unwired: 1 out]
                    }
                  }
                }
                frame True {
                  n178 = call "Is Value Changed.vim"("value"=w458) -> ("changed or first call?"=w457:bool)
                  n179 = Enqueue Element(queue=w450, element=modesEnum."Idle" ("modesEnum")) -> (queue out=w449:refnum<queue>)  [unwired: 2 in, 2 out]
                  n180 = Concatenate Strings("STOP" ("write buffer"), "\n" ("write buffer")) -> (w451:string)
                  n181 = case shown="True" w457 {
                    tunnel: w451 -> [_ w464]
                    tunnel: w459 -> [_ w463]
                    tunnel: [_ w462] -> w456
                    tunnel: w455 -> [_ w461]
                    tunnel: [_ w460] -> w454
                    frame False {
                    }
                    frame True {
                      n182 = VISA Write(VISA resource name=w463, write buffer=w464, error in (no error)=w461) -> (VISA resource name out=w462:refnum<visa-resource-name>, error out=w460:errorcluster)  [unwired: 1 out]
                    }
                  }
                }
              }
              "SafetyClose" <- TRUE
            }
            frame "SaveFile" {
              w467 = "%#g"
              w479 = string[][] []
              # "PID"
              # "ducer"
              # "Pad arrays to same size"
              # "blanks"
              # "Spike Position"
              n183 = Array Size(array=w481) -> (size(s)=w501:i32)
              n184 = Array Size(array=w497) -> (size(s)=w468:i32)
              n185 = disable-structure shown="Disabled" {
                disable-tunnel: w468 -> [w515 _]
                frame Disabled {
                  n186 = for {
                    N: w515 -> [_]
                    n187 = Number To Fractional String() -> ()  [unwired: 4 in, 1 out]
                  }
                }
                frame Enabled {
                }
              }
              n188 = Max & Min(x=w468, y=w501) -> (max(x,y)=w504:i32)  [unwired: 1 out]
              n189 = Array Size(array=w480) -> (size(s)=w503:i32)
              n190 = Max & Min(x=w504, y=w503) -> (max(x,y)=w502:i32)  [unwired: 1 out]
              n191 = Subtract(x=w501, y=w502) -> (x-y=w491:i32)
              n192 = Subtract(x=w502, y=w468) -> (x-y=w499:i32)
              n193 = Subtract(x=w502, y=w503) -> (x-y=w490:i32)
              n194 = Array To Spreadsheet String(array=w481, 3:w467) -> (spreadsheet string=w482:string)  [unwired: 1 in]
              n195 = Get Date/Time In Seconds() -> (seconds since 1Jan1904=w484:timestamp)
              n196 = Array To Spreadsheet String(delimiter (Tab)=",", array=w497, 3:w467) -> (spreadsheet string=w466:string)
              "spike str" <- w466
              n197 = Seconds To Date/Time(time stamp (now)=w484) -> ()  [unwired: 1 in, 1 out]
              n198 = Array To Spreadsheet String(array=w480, 3:w467) -> (spreadsheet string=w511:string)  [unwired: 1 in]
              n199 = Initialize Array("", w491) -> (w494:string[])
              n200 = Initialize Array("", w499) -> (w498:string[])
              n201 = Format Date/Time String(time format string (%c)="%Y-%m-%d_%H-%M-%S", seconds (now)=w484) -> (date/time string=w486:string)  [unwired: 1 in]
              n202 = Spreadsheet String To Array(format string=w467, spreadsheet string=w511, array type (2D Dbl)=w479) -> (array=w469:string[][])  [unwired: 1 in]
              "Array-to-save PID" <- w469
              n203 = Spreadsheet String To Array(format string=w467, spreadsheet string=w482, array type (2D Dbl)=w479) -> (array=w470:string[][])  [unwired: 1 in]
              "Array-to-save Pressure" <- w470
              n204 = Spreadsheet String To Array(format string=w467, spreadsheet string=w466, array type (2D Dbl)=w479) -> (array=w471:string[][])  [unwired: 1 in]
              "Array-to-save Spike" <- w471
              n205 = Initialize Array("", w490) -> (w492:string[])
              n206 = Build Array (concatenate)(w470, w494) -> (w489:string[][])
              n207 = Build Array (concatenate)(w469, w492) -> (w488:string[][])
              n208 = Build Array (concatenate)(w471, w498) -> (w496:string[][])
              n209 = Concatenate Strings("/needleValveData_", w486) -> (w474:string)
              n210 = call "File Dialog"("prompt"="Please Select Folder for Graph Data to be Saved", "default name"=w474) -> ("selected path"=w477:path)  [unwired: 10 in, 3 out]
              n211 = Array Size(array=w496) -> (size(s)=w507:i32[])
              n212 = Path To String(path=w477) -> (string=w475:string)
              n213 = Index Array(array=w507, index=0) -> (element=w505:i32)
              n214 = Concatenate Strings(w475, w474, ".csv") -> (w478:string)
              n215 = Initialize Array("", w505, 1) -> (w512:string[][])
              n216 = Build Array (concatenate)(string[] ["", "Time", "Spike Position", " ", "", "Time", "Pressure Ducer", "", "", "Time", "PID Output"], w496, w512, w512, w489, w512, w512, w488) -> (w472:string[][])
              "Array-to-save" <- w472
              n217 = String To Path(string=w478) -> (path=w476:path)
              "to save" <- w476
              n218 = call-poly <vilib>:"Write Delimited Spreadsheet.vi"("file path (dialog if empty)"=w476, "2D data"=w472, "delimiter (\\t)"=",") -> ()  [unwired: 11 in, 2 out]
            }
          }
          "Spike Position \n(via Potentiometer)" <- w56
          "distance to go" <- w67
          "spike position" <- w60
          "Idle" <- w65
          n219 = event shown="[1] \"Set setPoint\": Value Change" {
            selector: _ -> [_ _ _]
            dyn-events: _ -> [_ _ _]
            timeout: w54 -> [_ _ _]
            tunnel: [_ w94 w95] -> w55
            event Timeout {
              n220 = event-data() -> ()  [unwired: 1 in, 3 out]
            }
            event "Set setPoint": Value Change {
              n221 = event-data() -> ("NewVal"=w94:dbl)  [unwired: 1 in, 5 out]
            }
            event "setPoint": Value Change {
              n222 = event-data() -> ("NewVal"=w95:dbl)  [unwired: 1 in, 5 out]
            }
          }
          n223 = event shown="[0] \"AutoTune PID Params\": Value Change" {
            selector: _ -> [_ _ _ _]
            dyn-events: _ -> [_ _ _ _]
            timeout: w54 -> [_ _ _ _]
            tunnel: [_ w97 w98 _] -> w58
            event "AutoTune PID Params": Value Change {
              n224 = event-data() -> ("NewVal"=w96:bool)  [unwired: 1 in, 5 out]
              n225 = property on="Autotune" class="Bool (strict)"("Value"=w96) -> ()  [unwired: 2 in, 2 out]
            }
            event "Set Spike Position (in)": Value Change {
              n226 = event-data() -> ("NewVal"=w97:dbl)  [unwired: 1 in, 5 out]
            }
            event "Set Spike Position": Value Change {
              n227 = event-data() -> ("NewVal"=w98:dbl)  [unwired: 1 in, 5 out]
            }
            event Timeout {
              n228 = event-data() -> ()  [unwired: 1 in, 3 out]
            }
          }
          n229 = VISA Read(VISA resource name=w52, byte count=16, error in (no error)=w49) -> (VISA resource name out=w51:refnum<visa-resource-name>, read buffer=→"Motor Response":string, error out=w48:errorcluster)  [unwired: 1 out]
          "Set Motor RPM" <- "?"
          "Motor Signal" <- w87
          "the set position" <- w59
          "the setted point" <- w57
        }
        n230 = call "LJM_OpenS.vi"() -> ("error out"=w41:errorcluster, "Handle"=w45:i32)  [unwired: 10 in]
        n231 = Obtain Queue(element data type=enum16{"Start sensors", "load Values", "Idle"}."Start sensors" ("Enum")) -> (queue out=w37:refnum<queue>)  [unwired: 4 in, 2 out]
        n232 = call "LJM_GetHandleInfo.vi"("error in"=w41, "Handle In"=w45) -> ("error out"=w40:errorcluster, "ConnectionType"=→"ConnectionType":i32, "DeviceType"=→"DeviceType":i32, "Handle Out"=w32:i32, "Port"=→"Port":i32)  [unwired: 2 in, 3 out]
        n233 = Enqueue Element(queue=w37, element=enum16{"Start sensors", "load Values", "Idle"}."Idle" ("Enum")) -> (queue out=w36:refnum<queue>)  [unwired: 2 in, 2 out]
        n234 = call "LJM_eWriteNames.vi"("Handle In"=w32, "aNames"=string[] ["AIN0_RANGE", "AIN3_RANGE", "AIN2_EF_CONFIG_A", "AIN2_EF_INDEX", "AIN4_RANGE"], "aValuesIn"=dbl[] [10.0, 10.0, 0.0, 22.0, 10.0]) -> ("Handle Out"=w31:i32)  [unwired: 10 in, 2 out]
        n235 = while {
          tunnel: w40 -> [w532]
          tunnel: [w531] -> w39
          tunnel: w31 -> [w530]
          tunnel: [w529] -> w38
          tunnel: w36 -> [w528]
          tunnel: [w525] -> w34
          shift-right: [w519] -> _
          shift-left: _ -> [w518]
          stop <- "loop stop 1" stop-if-true
          n236 = Dequeue Element(queue=w528) -> (queue out=w526:refnum<queue>, element=w527:enum16{"Start sensors", "load Values", "Idle"})  [unwired: 2 in, 2 out]
          n237 = Wait Until Next ms Multiple(millisecond multiple="Sensor Loop Rate (ms)") -> (millisecond timer value=w524:u32)
          n238 = case shown="\"Start sensors\"" w527 {
            tunnel: w532 -> [_ _ w604]
            tunnel: [_ _ w603] -> w531
            tunnel: w530 -> [_ _ w606]
            tunnel: [_ _ w605] -> w529
            tunnel: w526 -> [w535 w558 w611]
            tunnel: [w534 w557 w610] -> w525
            tunnel: [_ _ w598] -> _
            tunnel: "Sensor Offsets" -> [_ _ w600]
            tunnel: "Sensor K-values" -> [_ _ w599]
            tunnel: [_ _ w592] -> w519
            tunnel: w518 -> [_ _ w591]
            tunnel: "Sensor Loop Rate (ms)" -> [_ _ _]
            frame "load Values" {
              n239 = flat-sequence {
                frame #0 {
                  n240 = Two Button Dialog(message="Sensor and RPM File Selection" ("Message")) -> (T button?=w536:bool)  [unwired: 2 in]
                  n241 = case shown="False" w536 {
                    frame False {
                    }
                    frame True {
                      # "Loading Motor RPM"
                      n242 = call-poly <vilib>:"Read Delimited Spreadsheet.vi"() -> ("all rows"=w539:dbl[][])  [unwired: 10 in, 5 out]
                      n243 = Index Array(array=w539, index (row)=1) -> (element=w551:dbl[])  [unwired: 1 in]
                      n244 = Index Array(array=w539, index (row)=3) -> (element=w545:dbl[])  [unwired: 1 in]
                      n245 = Index Array(array=w539, index (row)=0) -> (element=w553:dbl[])  [unwired: 1 in]
                      n246 = Index Array(array=w539, index (row)=2) -> (element=w549:dbl[])  [unwired: 1 in]
                      n247 = Index Array(array=w539, index (row)=4) -> (element=w541:dbl[])  [unwired: 1 in]
                      n248 = property on="Sensor Offsets" class="Arr (strict)"("Value"=w551) -> ()  [unwired: 2 in, 2 out]
                      n249 = property on="Sensor K-values" class="Arr (strict)"("Value"=w553) -> ()  [unwired: 2 in, 2 out]
                      n250 = Index Array(array=w545, index=0) -> (element=w543:dbl)
                      n251 = Index Array(array=w541, index=0) -> (element=w538:dbl)
                      n252 = Index Array(array=w549, index=0) -> (element=w547:dbl)
                      n253 = property on="Sensor Loop Rate (ms)" class="DigNum (strict)"("Value"=w543) -> ()  [unwired: 2 in, 2 out]
                      n254 = property on="Motor Control Loop Rate (ms)" class="DigNum (strict)"("Value"=w538) -> ()  [unwired: 2 in, 2 out]
                      n255 = property class="DigNum (strict)"("Value"=w547) -> ()  [unwired: 2 in, 2 out]
                    }
                  }
                }
                frame #1 {
                }
                frame #2 {
                }
              }
              n256 = Enqueue Element(queue=w535, element=enum16{"Start sensors", "load Values", "Idle"}."Idle" ("Enum")) -> (queue out=w534:refnum<queue>)  [unwired: 2 in, 2 out]
            }
            frame "Idle" {
              w556 = T3."Enabled" ("Disabled")
              n257 = event shown="[3] \"Use Dummy Data\": Value Change" {
                selector: _ -> [_ _ _ _]
                dyn-events: _ -> [_ _ _ _]
                timeout: _ -> [_ _ _ _]
                tunnel: w558 -> [w561 w564 w567 w569]
                tunnel: [w560 w563 w566 w568] -> w557
                event "Save Inputs": Value Change {
                  n258 = event-data() -> ()  [unwired: 1 in, 6 out]
                  n259 = Enqueue Element(queue=w561, element=enum16{"Start sensors", "load Values", "Idle"}."Idle" ("Enum")) -> (queue out=w560:refnum<queue>)  [unwired: 2 in, 2 out]
                }
                event "Load Inputs": Value Change {
                  n260 = event-data() -> ()  [unwired: 1 in, 6 out]
                  n261 = Enqueue Element(queue=w564, element=enum16{"Start sensors", "load Values", "Idle"}."Idle" ("Enum")) -> (queue out=w563:refnum<queue>)  [unwired: 2 in, 2 out]
                }
                event "Start Sensors": Value Change {
                  n262 = event-data() -> ()  [unwired: 1 in, 6 out]
                  n263 = Enqueue Element(queue=w567, element=enum16{"Start sensors", "load Values", "Idle"}."Start sensors" ("Enum")) -> (queue out=w566:refnum<queue>)  [unwired: 2 in, 2 out]
                }
                event "Use Dummy Data": Value Change {
                  n264 = event-data() -> ()  [unwired: 1 in, 6 out]
                  n265 = Enqueue Element(queue=w569, element=enum16{"Start sensors", "load Values", "Idle"}."Start sensors" ("Enum")) -> (queue out=w568:refnum<queue>)  [unwired: 2 in, 2 out]
                }
              }
              n266 = property on="Start Sensors" class="Bool"("DisabledEnum"=w556) -> ()  [unwired: 2 in, 2 out]
              n267 = property on="Save Inputs" class="Bool"("DisabledEnum"=w556) -> ()  [unwired: 2 in, 2 out]
              n268 = property on="Load Inputs" class="Bool"("DisabledEnum"=w556) -> ()  [unwired: 2 in, 2 out]
              n269 = property on="Stop Sensors" class="Bool"("DisabledEnum"=T3."Disabled and Grayed Out" ("Disabled")) -> ()  [unwired: 2 in, 2 out]
            }
            frame "Start sensors" {
              w572 = 50.0
              w608 = T3."Disabled and Grayed Out" ("Disabled")
              # "threshold"
              # "Sensor Calibration and LabJack Read"
              n270 = Array Size(array=w600) -> (size(s)=w601:i32)
              n271 = event shown="[3] Timeout" {
                selector: _ -> [_ _ _ _]
                dyn-events: _ -> [_ _ _ _]
                timeout: 50 -> [_ _ _ _]
                event "Use Avg": Value Change {
                  n272 = event-data() -> ("NewVal"=w612:bool)  [unwired: 1 in, 5 out]
                  n273 = case shown="True" w612 {
                    frame False {
                    }
                    frame True {
                      n274 = property on="Ducer1" class="Bool (strict)"("Value"=FALSE) -> ()  [unwired: 2 in, 2 out]
                      n275 = property on="Ducer2" class="Bool (strict)"("Value"=FALSE) -> ()  [unwired: 2 in, 2 out]
                      n276 = property on="Avg Ducers" class="Bool (strict)"("Value"=TRUE) -> ()  [unwired: 2 in, 2 out]
                    }
                  }
                }
                event "Use D2": Value Change {
                  n277 = event-data() -> ("NewVal"=w616:bool)  [unwired: 1 in, 5 out]
                  n278 = case shown="True" w616 {
                    frame False {
                    }
                    frame True {
                      n279 = property on="Ducer1" class="Bool (strict)"("Value"=FALSE) -> ()  [unwired: 2 in, 2 out]
                      n280 = property on="Ducer2" class="Bool (strict)"("Value"=TRUE) -> ()  [unwired: 2 in, 2 out]
                      n281 = property on="Avg Ducers" class="Bool (strict)"("Value"=FALSE) -> ()  [unwired: 2 in, 2 out]
                    }
                  }
                }
                event "Use D1": Value Change {
                  n282 = event-data() -> ("NewVal"=w620:bool)  [unwired: 1 in, 5 out]
                  n283 = case shown="True" w620 {
                    frame False {
                    }
                    frame True {
                      n284 = property on="Ducer1" class="Bool (strict)"("Value"=TRUE) -> ()  [unwired: 2 in, 2 out]
                      n285 = property on="Ducer2" class="Bool (strict)"("Value"=FALSE) -> ()  [unwired: 2 in, 2 out]
                      n286 = property on="Avg Ducers" class="Bool (strict)"("Value"=FALSE) -> ()  [unwired: 2 in, 2 out]
                    }
                  }
                }
                event Timeout {
                  n287 = event-data() -> ()  [unwired: 1 in, 3 out]
                }
              }
              n288 = property on="Stop Sensors" class="Bool"("DisabledEnum"=T3."Enabled" ("Disabled")) -> ()  [unwired: 2 in, 2 out]
              n289 = call "LJM_eReadNames.vi"("Handle In"=w606, "aNames"=string[] ["AIN0", "AIN3", "AIN2_EF_READ_A", "AIN4"], "error in"=w604) -> ("Handle Out"=w605:i32, "aValuesOut"=w596:dbl[], "error out"=w603:errorcluster)  [unwired: 9 in, 1 out]
              n290 = property on="Save Inputs" class="Bool"("DisabledEnum"=w608) -> ()  [unwired: 2 in, 2 out]
              n291 = property on="Start Sensors" class="Bool"("DisabledEnum"=w608) -> ()  [unwired: 2 in, 2 out]
              n292 = property on="Load Inputs" class="Bool"("DisabledEnum"=w608) -> ()  [unwired: 2 in, 2 out]
              n293 = for {
                N: w601 -> [_]
                tunnel: w600 -> [w633] mode=indexing
                tunnel: w599 -> [w634] mode=indexing
                tunnel: w596 -> [w636] mode=indexing
                tunnel: [w632] -> w585 mode=indexing
                n294 = Multiply(x=w634, y=w636) -> (x*y=w635:dbl)
                n295 = Add(x=w633, y=w635) -> (x+y=w632:dbl)
              }
              n296 = Array Size(array=w585) -> (size(s)=w595:i32)
              n297 = Index Array(array=w585, index=T4."Potentiometer" ("labjacksInputs")) -> (element=w598:dbl)
              "Potentiometer distance" <- w598
              n298 = Index Array(array=w585, index=T4."Thermocouple" ("labjacksInputs")) -> (element=→"?" →"Stagnation Flow Temp (K)\n(For Refrence only)":dbl)
              n299 = for {
                N: w595 -> [_]
                tunnel: w585 -> [w631] mode=indexing
                tunnel: [w629] -> w594 mode=indexing
                n300 = Number To Decimal String(number=w631, width (-)=i16 5) -> (decimal integer string=w629:string)
              }
              n301 = Index Array(array=w585, index=T4."Ducer2" ("labjacksInputs")) -> (element=w575:dbl)
              "Raw Pressure Ducer 2" <- w575
              n302 = Index Array(array=w585, index=T4."Ducer" ("labjacksInputs")) -> (element=w573:dbl)
              "Raw Pressure Ducer" <- w573
              n303 = Subtract(x=w575, y=w573) -> (x-y=w583:dbl)
              n304 = Add(x=w575, y=w573) -> (x+y=w580:dbl)
              n305 = Absolute Value(x=w583) -> (abs(x)=w582:dbl)
              n306 = Format Date/Time String(time format string (%c)="%H%M%S%3u") -> (date/time string=w589:string)  [unwired: 2 in]
              n307 = Divide(x=w580, y=2) -> (x/y=w574:dbl)
              n308 = Insert Into Array(array=w594, new element=w589) -> (w593:string[])  [unwired: 1 in]
              n309 = In Range and Coerce(upper limit=w572, x=w582, lower limit=w572) -> ()  [unwired: 2 out]
              n310 = case shown="False" "Use Avg" {
                tunnel: [w624 w628] -> w579
                tunnel: "Use D2" -> [_ _]
                tunnel: "Use D1" -> [w627 _]
                tunnel: w575 -> [w625 _]
                tunnel: w574 -> [_ w628]
                tunnel: w573 -> [w626 _]
                frame False {
                  n311 = Select(t=w625, s=w627, f=w626) -> (s? t:f=w624:dbl)
                }
                frame True {
                }
              }
              "Read Pressure Ducer" <- w579
              n312 = Build Array (concatenate)(w593, w591) -> (w592:string[][])
              n313 = case shown="False" "Stop Sensors" {
                tunnel: w611 -> [w639 w642]
                tunnel: [w638 w641] -> w610
                frame False {
                  n314 = Enqueue Element(queue=w639, element=enum16{"Start sensors", "load Values", "Idle"}."Start sensors" ("Enum")) -> (queue out=w638:refnum<queue>)  [unwired: 2 in, 2 out]
                }
                frame True {
                  n315 = Enqueue Element(queue=w642, element=enum16{"Start sensors", "load Values", "Idle"}."Idle") -> (queue out=w641:refnum<queue>)  [unwired: 2 in, 2 out]
                }
              }
            }
          }
          n316 = Divide(x=w524, y=u32 1000) -> (x/y=→"Time Since Start (s)\n(For Reference Only)":dbl)
        }
        n317 = Release Queue(queue=w34) -> ()  [unwired: 2 in, 3 out]
        n318 = call "LJM_Close.vi"("error in"=w39, "Handle"=w38) -> ("error out"=→"Labjack error":errorcluster)  [unwired: 9 in]
        n319 = Release Queue(queue=w26) -> ()  [unwired: 2 in, 3 out]
        n320 = VISA Close(VISA resource name=w22, error in (no error)=w21) -> (error out=→"Arduino Error":errorcluster)
      }
      frame "IdleControllers", Default {
        n321 = property on="Connect" class="Bool (strict)"() -> ("Value"=w645:bool)  [unwired: 2 in, 2 out]
        n322 = case shown="False" w645 {
          tunnel: w643 -> [w648 w650]
          tunnel: [w647 w649] -> w644
          frame False {
            n323 = Enqueue Element(queue=w648, element=ControllerModeEnum."IdleControllers" ("ControllerModeEnum")) -> (queue out=w647:refnum<queue>)  [unwired: 2 in, 2 out]
          }
          frame True {
            n324 = Enqueue Element(queue=w650, element=ControllerModeEnum."startControllers" ("ControllerModeEnum")) -> (queue out=w649:refnum<queue>)  [unwired: 2 in, 2 out]
          }
        }
      }
    }
    n325 = And(x="Connect", y="Disconnect") -> (x .and. y?=w8:bool)
  }
